vi "initCSMs.vi"(7 "Enable building lvlibp?":bool, 8 "error in (no error)":errorcluster, 11 "TestCase in":refnum<class "testcase-CSMNonCSMCallerSupportAPI.lvclass">) -> (0 "error out":errorcluster, 3 "TestCase out":refnum<class "testcase-CSMNonCSMCallerSupportAPI.lvclass">)   [LabVIEW 2017, in "testcase-CSMNonCSMCallerSupportAPI.lvclass"]
uses:
  testcase-CSMNonCSMCallerSupportAPI.lvclass
  testcase-CSMNonCSMCallerSupportAPI.lvclass/testcase-CSMNonCSMCallerSupportAPI.ctl
  CSM/Normal-CSM.vi
  <vilib>/AppBuilder/AB_API_Simple/Build (path).vi
  CSM/Chain1.vi
  CSM/Chain2.vi
  CSM/Chain3.vi
  <vilib>/addons/_JKI Toolkits/VI Tester/TestCase.llb/TestCase.lvclass
  CSM/CSM-Testcase.lvlib
  src/user.lib/_NEVSTOP/Communicable State Machine(CSM)/Communicable State Machine.lvlib
  <vilib>/AppBuilder/AB_API_Simple/NI_App_Builder_API.lvlib
  C:/Program Files (x86)/National Instruments/LabVIEW 2017/vi.lib/addons/_JKI Toolkits/VI Tester/TestCase.llb/TestCase.lvclass
panel:
  out "Waited (ms)":u32
  out "CSMs Left":string[](array[string])
  out "Generated files":path[](array[path])
  out "CSMs":string[](array[string])
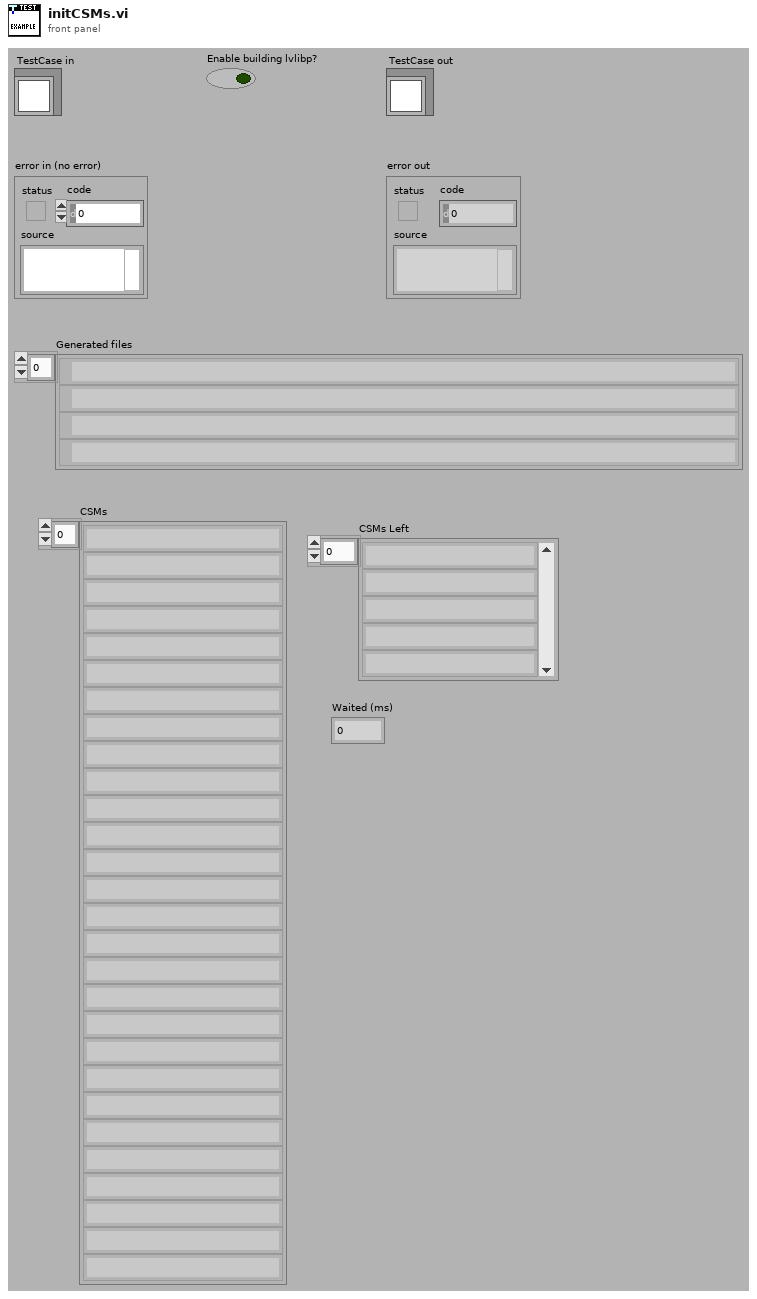
[diagram p1: front panel]
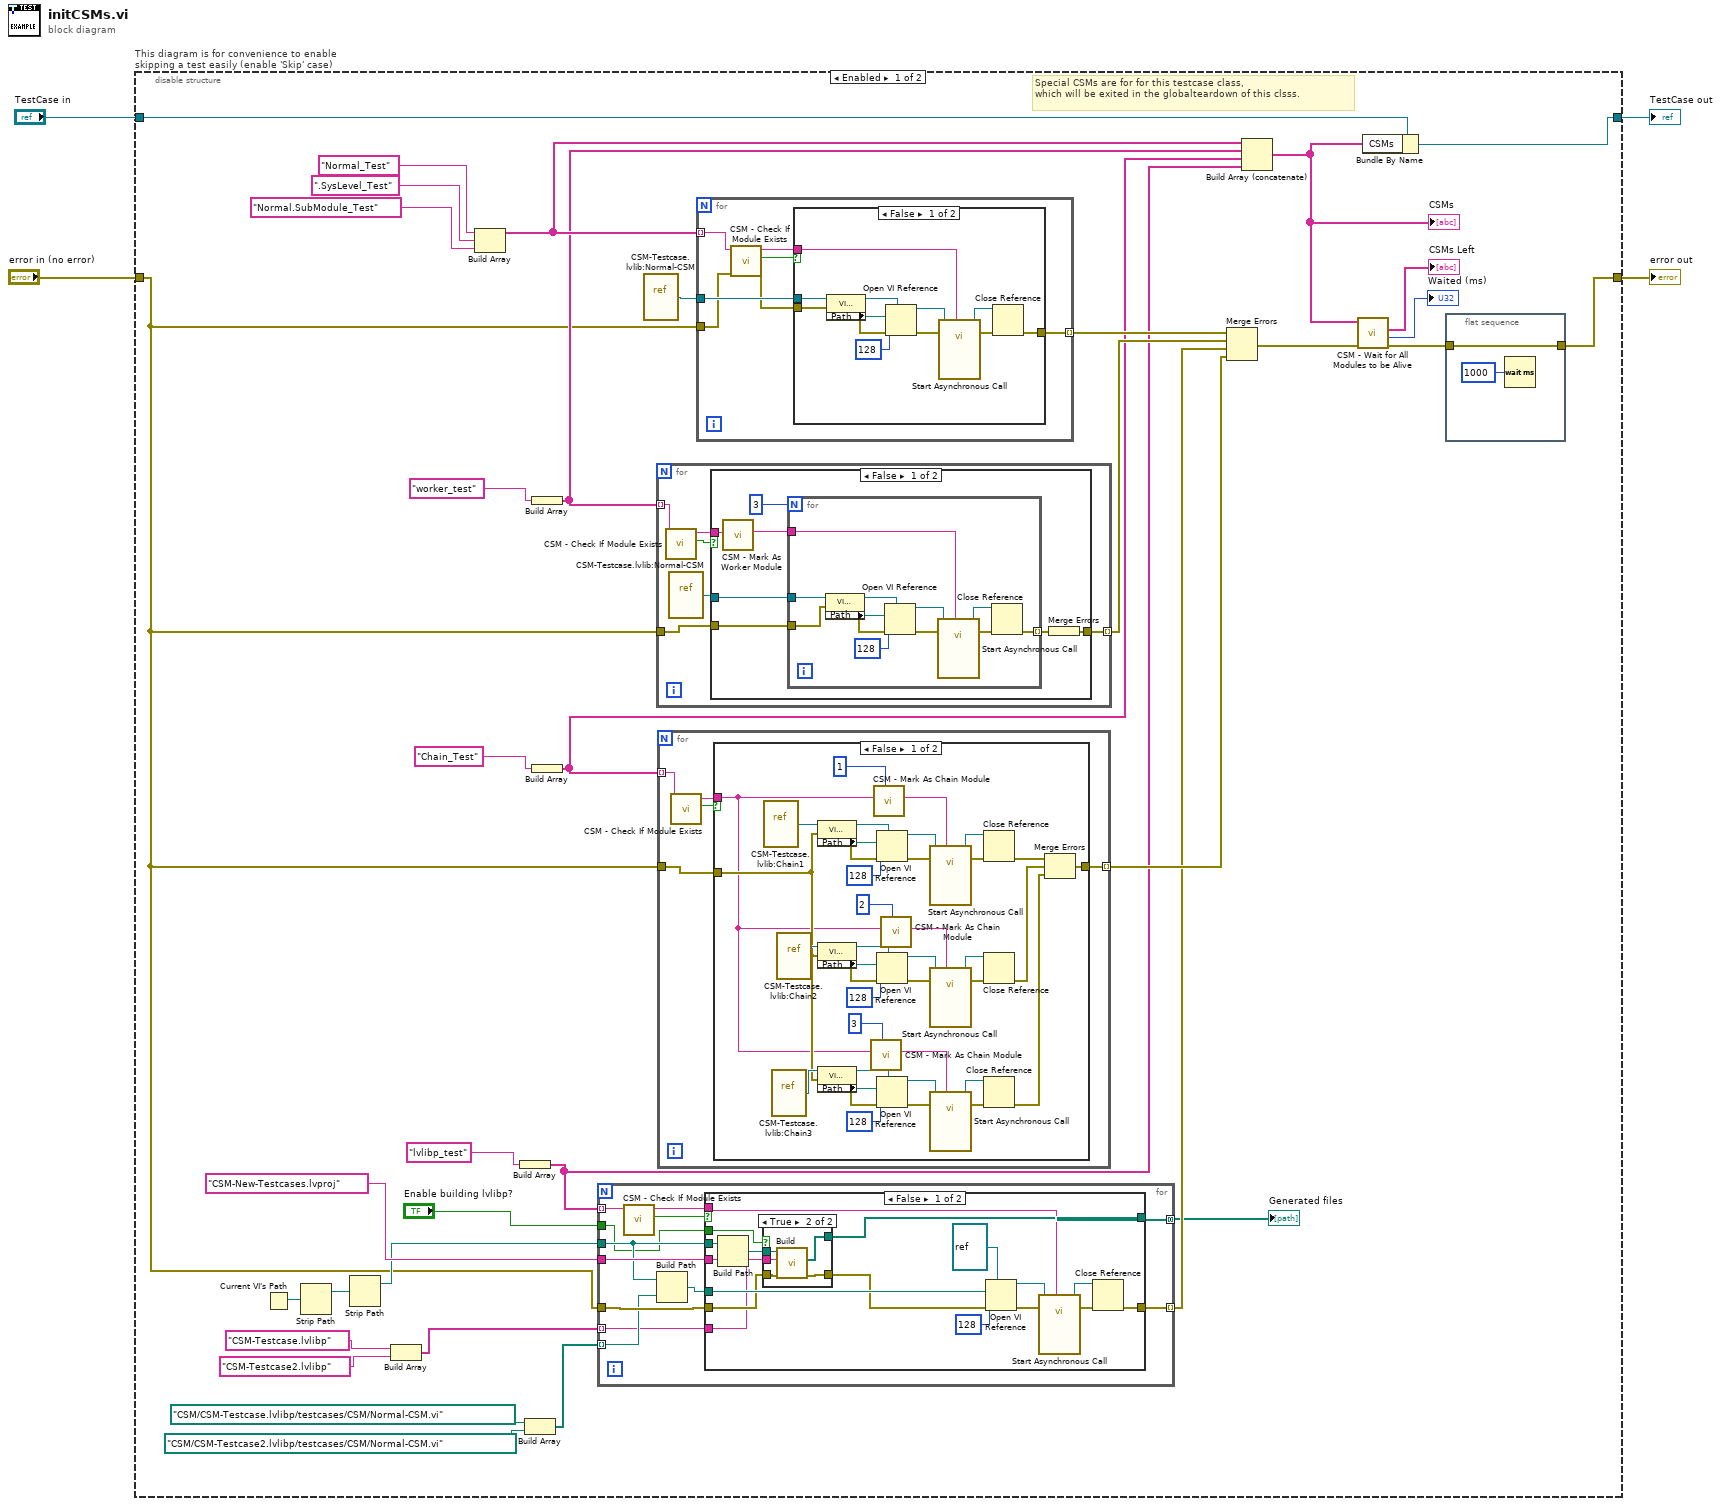
[diagram p0: block diagram]
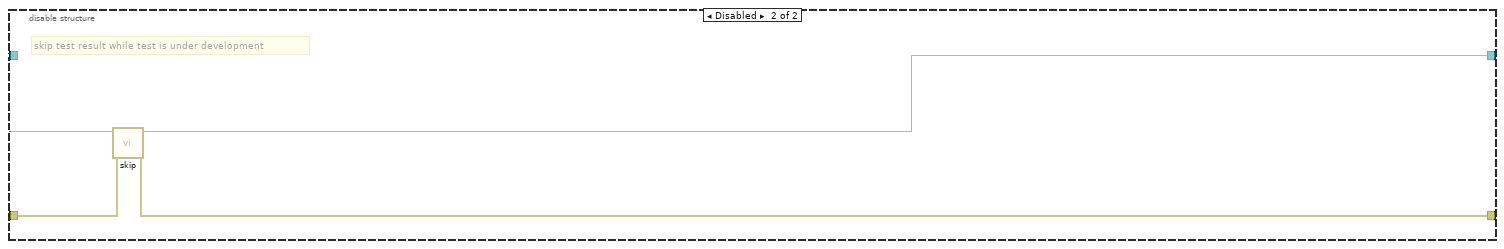
[diagram p7: hidden frame]
diagram:
  n1 = disable-structure "This diagram is for convenience to enable skipping a test easily (enable 'Skip' case)" shown="Enabled" {
    disable-tunnel: "TestCase in" -> [w9 w173]
    disable-tunnel: [w7 w171] -> w1
    disable-tunnel: [w6 w172] -> w3
    disable-tunnel: "error in (no error)" -> [w10 w170]
    frame Enabled {
      # "Special CSMs are for for this testcase class,\nwhich will be exited in the globalteardown of this clsss."
      n2 = Current VI's Path() -> (path=w36:path)
      n3 = Strip Path(path=w36) -> (stripped path=w37:path)  [unwired: 1 out]
      n4 = Strip Path(path=w37) -> (stripped path=w38:path)  [unwired: 1 out]
      n5 = Build Array("CSM-Testcase.lvlibp" ("Name of build specification (if empty: build all)"), "CSM-Testcase2.lvlibp" ("Name of build specification (if empty: build all)")) -> (w16:string[])
      n6 = Build Array("Normal_Test" ("Name (\"\" to Use UUID)"), ".SysLevel_Test" ("Name (\"\" to Use UUID)"), "Normal.SubModule_Test" ("Name (\"\" to Use UUID)")) -> (w32:string[])
      n7 = Build Array("lvlibp_test" ("Name (\"\" to Use UUID)")) -> (w22:string[])
      n8 = Build Array(path "CSM/CSM-Testcase.lvlibp/testcases/CSM/Normal-CSM.vi" ("vi path"), path "CSM/CSM-Testcase2.lvlibp/testcases/CSM/Normal-CSM.vi" ("vi path")) -> (w19:path[])
      n9 = Build Array("worker_test" ("Name (\"\" to Use UUID)")) -> (w26:string[])
      n10 = Build Array("Chain_Test" ("Name (\"\" to Use UUID)")) -> (w24:string[])
      n11 = for {
        tunnel: "CSM-New-Testcases.lvproj" ("name or relative path") -> [w52]
        tunnel: w38 -> [w47]
        tunnel: w22 -> [w49] mode=indexing
        tunnel: w19 -> [w48] mode=indexing
        tunnel: w16 -> [w45] mode=indexing
        tunnel: [w44] -> w15 mode=concatenating
        tunnel: "Enable building lvlibp?" -> [w43]
        tunnel: w10 -> [w53]
        tunnel: [w51] -> w35 mode=indexing
        n12 = call "CSM - Check If Module Exists.vi"("CSM Name"=w49) -> ("Exist?"=w54:bool, "CSM Name (Dup)"=w50:string)  [unwired: 8 in, 1 out]
        n13 = Build Path(base path=w47, name or relative path=w48) -> (appended path=w46:path)
        n14 = case shown="False" w54 {
          tunnel: [w71 w78] -> w51
          tunnel: w46 -> [w64 _]
          tunnel: w47 -> [w63 _]
          tunnel: w52 -> [w61 _]
          tunnel: w50 -> [w60 _]
          tunnel: w53 -> [w59 w78]
          tunnel: w45 -> [w57 _]
          tunnel: [w56 _] -> w44
          tunnel: w43 -> [w55 _]
          frame False {
            n15 = Build Path(base path=w63, name or relative path=w61) -> (appended path=w62:path)
            n16 = case shown="True" w55 {
              tunnel: w62 -> [_ w77]
              tunnel: w59 -> [w72 w76]
              tunnel: [w72 w75] -> w58
              tunnel: w57 -> [_ w74]
              tunnel: [_ w73] -> w56
              frame False {
              }
              frame True {
                n17 = call-poly <vilib>:"Build.vi"("error in (no error)"=w76, "Name of build specification (if empty: build all)"=w74, "Path to project"=w77) -> ("error out"=w75:errorcluster, "Generated files"=w73:path[])  [unwired: 7 in]
              }
            }
            n18 = Open VI Reference(type specifier VI Refnum (for type only)=refnum<vi> refnum ("reference out"), vi path=w64, options=128, error in (no error)=w58) -> (vi reference=w67:refnum<vi>, error out=w69:errorcluster)  [unwired: 2 in]
            n19 = call-by-ref "Start Asynchronous Call"(reference=w67, error in=w69, "Name (\"\" to Use UUID)"=w60) -> (reference out=w66:refnum<vi>, error out=w68:errorcluster)  [unwired: 11 in]
            n20 = Close Reference(reference=w66, error in (no error)=w68) -> (error out=w71:errorcluster)
          }
          frame True {
          }
        }
      }
      "Generated files" <- w15
      n21 = vi-ref "CSM-Testcase.lvlib:Normal-CSM.vi"() -> (w28:refnum<vi>)
      n22 = for {
        tunnel: w26 -> [w125] mode=indexing
        tunnel: w10 -> [w129]
        tunnel: [w126] -> w34 mode=indexing
        n23 = call "CSM - Check If Module Exists.vi"("CSM Name"=w125) -> ("Exist?"=w128:bool, "CSM Name (Dup)"=w127:string)  [unwired: 8 in, 1 out]
        n24 = vi-ref "CSM-Testcase.lvlib:Normal-CSM.vi"() -> (w124:refnum<vi>)
        n25 = case shown="False" w128 {
          tunnel: w124 -> [w136 _]
          tunnel: [w130 w149] -> w126
          tunnel: w129 -> [w132 w149]
          tunnel: w127 -> [w131 _]
          frame False {
            n26 = call "CSM - Mark As Worker Module.vi"("CSM Name"=w131) -> ("CSM Name (Marked As Worker)"=w133:string)  [unwired: 9 in]
            n27 = for {
              N: 3 -> [_]
              tunnel: w136 -> [w140]
              tunnel: w133 -> [w139]
              tunnel: [w138] -> w134 mode=indexing
              tunnel: w132 -> [w137]
              n28 = property class="VI (strict)"(reference=w140, error in=w137) -> (reference out=w146:refnum<vi>, error out=w144:errorcluster, "Path"=w143:path)
              n29 = Open VI Reference(type specifier VI Refnum (for type only)=w146, vi path=w143, options=128, error in (no error)=w144) -> (vi reference=w142:refnum<vi>, error out=w147:errorcluster)  [unwired: 2 in]
              n30 = call-by-ref "Start Asynchronous Call"(reference=w142, error in=w147, "Name (\"\" to Use UUID)"=w139) -> (reference out=w141:refnum<vi>, error out=w145:errorcluster)  [unwired: 11 in]
              n31 = Close Reference(reference=w141, error in (no error)=w145) -> (error out=w138:errorcluster)
            }
            n32 = Merge Errors(w134) -> (w130:errorcluster)
          }
          frame True {
          }
        }
      }
      n33 = for {
        tunnel: w24 -> [w79] mode=indexing
        tunnel: w10 -> [w83]
        tunnel: [w81] -> w40 mode=indexing
        n34 = call "CSM - Check If Module Exists.vi"("CSM Name"=w79) -> ("Exist?"=w82:bool, "CSM Name (Dup)"=w80:string)  [unwired: 8 in, 1 out]
        n35 = case shown="False" w82 {
          tunnel: [w86 w123] -> w81
          tunnel: w83 -> [w85 w123]
          tunnel: w80 -> [w84 _]
          frame False {
            n36 = vi-ref "CSM-Testcase.lvlib:Chain1.vi"() -> (w122:refnum<vi>)
            n37 = vi-ref "CSM-Testcase.lvlib:Chain3.vi"() -> (w104:refnum<vi>)
            n38 = vi-ref "CSM-Testcase.lvlib:Chain2.vi"() -> (w105:refnum<vi>)
            n39 = property class="VI (strict)"(reference=w122, error in=w85) -> (reference out=w119:refnum<vi>, error out=w117:errorcluster, "Path"=w116:path)
            n40 = property class="VI (strict)"(reference=w105, error in=w85) -> (reference out=w108:refnum<vi>, error out=w110:errorcluster, "Path"=w111:path)
            n41 = property class="VI (strict)"(reference=w104, error in=w85) -> (reference out=w101:refnum<vi>, error out=w99:errorcluster, "Path"=w98:path)
            n42 = call "CSM - Mark As Chain Module.vi"("Order"=3, "CSM Name"=w84) -> ("CSM Name (Marked As Chain)"=w92:string)  [unwired: 8 in]
            n43 = call "CSM - Mark As Chain Module.vi"("Order"=1, "CSM Name"=w84) -> ("CSM Name (Marked As Chain)"=w90:string)  [unwired: 8 in]
            n44 = Open VI Reference(type specifier VI Refnum (for type only)=w119, vi path=w116, options=128, error in (no error)=w117) -> (vi reference=w115:refnum<vi>, error out=w120:errorcluster)  [unwired: 2 in]
            n45 = Open VI Reference(type specifier VI Refnum (for type only)=w108, vi path=w111, options=128, error in (no error)=w110) -> (vi reference=w112:refnum<vi>, error out=w107:errorcluster)  [unwired: 2 in]
            n46 = Open VI Reference(type specifier VI Refnum (for type only)=w101, vi path=w98, options=128, error in (no error)=w99) -> (vi reference=w97:refnum<vi>, error out=w102:errorcluster)  [unwired: 2 in]
            n47 = call "CSM - Mark As Chain Module.vi"("Order"=2, "CSM Name"=w84) -> ("CSM Name (Marked As Chain)"=w91:string)  [unwired: 8 in]
            n48 = call-by-ref "Start Asynchronous Call"(reference=w115, error in=w120, "Name (\"\" to Use UUID)"=w90) -> (reference out=w114:refnum<vi>, error out=w118:errorcluster)  [unwired: 11 in]
            n49 = call-by-ref "Start Asynchronous Call"(reference=w112, error in=w107, "Name (\"\" to Use UUID)"=w91) -> (reference out=w113:refnum<vi>, error out=w109:errorcluster)  [unwired: 11 in]
            n50 = call-by-ref "Start Asynchronous Call"(reference=w97, error in=w102, "Name (\"\" to Use UUID)"=w92) -> (reference out=w96:refnum<vi>, error out=w100:errorcluster)  [unwired: 11 in]
            n51 = Close Reference(reference=w114, error in (no error)=w118) -> (error out=w95:errorcluster)
            n52 = Close Reference(reference=w113, error in (no error)=w109) -> (error out=w94:errorcluster)
            n53 = Close Reference(reference=w96, error in (no error)=w100) -> (error out=w93:errorcluster)
            n54 = Merge Errors(w95, w94, w93) -> (w86:errorcluster)
          }
          frame True {
          }
        }
      }
      n55 = for {
        tunnel: w28 -> [w156]
        tunnel: w32 -> [w152] mode=indexing
        tunnel: [w155] -> w33 mode=indexing
        tunnel: w10 -> [w154]
        n56 = call "CSM - Check If Module Exists.vi"("Error In"=w154, "CSM Name"=w152) -> ("error out"=w153:errorcluster, "Exist?"=w150:bool, "CSM Name (Dup)"=w151:string)  [unwired: 7 in]
        n57 = case shown="False" w150 {
          tunnel: w156 -> [w160 _]
          tunnel: [w159 w169] -> w155
          tunnel: w153 -> [w158 w169]
          tunnel: w151 -> [w157 _]
          frame False {
            n58 = property class="VI (strict)"(reference=w160, error in=w158) -> (reference out=w166:refnum<vi>, error out=w164:errorcluster, "Path"=w163:path)
            n59 = Open VI Reference(type specifier VI Refnum (for type only)=w166, vi path=w163, options=128, error in (no error)=w164) -> (vi reference=w162:refnum<vi>, error out=w167:errorcluster)  [unwired: 2 in]
            n60 = call-by-ref "Start Asynchronous Call"(reference=w162, error in=w167, "Name (\"\" to Use UUID)"=w157) -> (reference out=w161:refnum<vi>, error out=w165:errorcluster)  [unwired: 11 in]
            n61 = Close Reference(reference=w161, error in (no error)=w165) -> (error out=w159:errorcluster)
          }
          frame True {
          }
        }
      }
      n62 = Merge Errors(w33, w34, w35, w40) -> (w14:errorcluster)
      n63 = Build Array (concatenate)(w32, w26, w24, w22) -> (w8:string[])
      "CSMs" <- w8
      n64 = call "CSM - Wait for All Modules to be Alive.vi"("Error In"=w14, "CSM Names"=w8) -> ("error out"=w5:errorcluster, "Waited (ms)"=→"Waited (ms)":u32, "CSMs Left"=→"CSMs Left":string[])  [unwired: 7 in]
      n65 = Bundle By Name(cluster=w9, "CSMs"=w8) -> (w7:refnum<class "testcase-CSMNonCSMCallerSupportAPI.lvclass">)
      n66 = flat-sequence {
        tunnel: [w41] -> w6
        tunnel: w5 -> [w41]
        frame #0 {
          n67 = Wait (ms)(milliseconds to wait=u32 1000) -> ()  [unwired: 1 out]
        }
      }
    }
    frame Disabled {
      # "skip test result while test is under development"
      n68 = call <vilib>:"skip.vi"("error in (no error)"=w170, "TestCase in"=w173) -> ("error out"=w172:errorcluster, "TestCase out"=w171:refnum<class "testcase-CSMNonCSMCallerSupportAPI.lvclass">)  [unwired: 8 in]
    }
  }
  "error out" <- w3
  "TestCase out" <- w1
